vi "ZM-HWM-helperAcquisition.vi"(8 "error in":errorcluster, 10 "Event Registration Refnum":refnum<event-registration>, 11 "ZM-HWM-hardware_manager in":refnum<class "ZM-HWM-hardware_manager.lvclass">) -> (0 "error out":errorcluster)   [LabVIEW 2020, in "ZM-HWM-hardware_manager.lvlib" / "ZM-HWM-hardware_manager.lvclass"]
doc: "Helper loop of the hardware manager, started by Actor Core beside Call Parent. Every interval (ms) it reads the hardware (ZM-HW-do), sends the package to its actor and plots test packages on the chart. It stops on the actor's stop event or on an error; on an error it sends Normal Stop to its own actor. Error-handling plan: none yet; an error stops this actor and, through its Last Ack, its caller."
uses:
  ZM-HWM-hardware_manager.lvclass
  ZM-HWM-hardware_manager.lvclass/ZM-HWM-hardware_manager.ctl
  common/ZM-PC-packages/ZM-PC-TP-test_package/ZM-PC-TP-test_package.lvclass
  common/ZM-CI-common_interfaces/ZM-CI-handlePackage Msg/ZM-CI-handlePackage Msg.lvclass
  <vilib>/ActorFramework/Stop Msg/Stop Msg.lvclass
  hardware/ZM-HW-hardware/ZM-HW-hardware/ZM-HW-hardware.lvclass
  <vilib>/ActorFramework/Message Enqueuer/Message Enqueuer.lvclass
  <vilib>/ActorFramework/Actor/Actor.lvclass
panel:
  out "interval measured (ms)":u32
  in  "interval set (ms)":u32=500
  out "live":cluster{"temperature_c":dbl, "duty_percent":dbl}(graph)
  in  "stop":bool
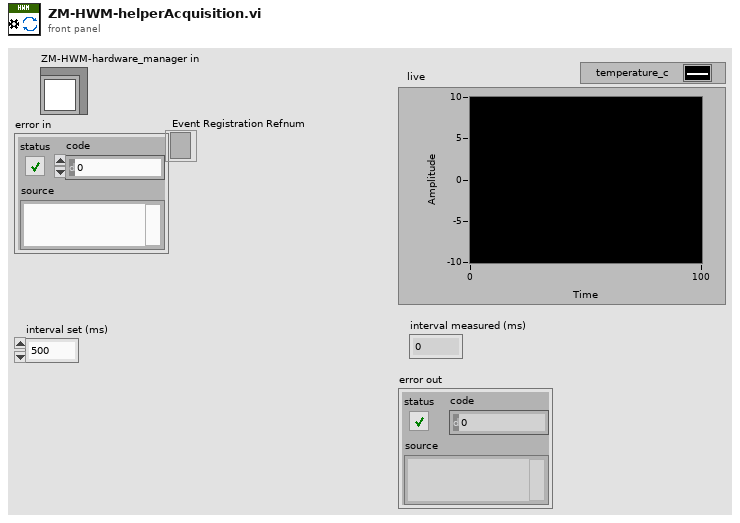
[diagram p1: front panel]
types:
  T1 = typedef "ZM-HWM-hardware_manager.lvlib/ZM-HWM-hardware_manager.lvclass/ZM-HWM-PRELAUNCH_SETTINGS.ctl" = cluster{"hardware":refnum<class "ZM-HW-hardware.lvclass">, "intervalMs":u32}
  T2 = typedef "ZM-PC-packages.lvlib/ZM-PC-TP-test_package.lvclass/ZM-PC-TP-DATA.ctl" = cluster{"temperature_c":dbl, "sample_index":i32, "duty_percent":u8, "sensor_ok":bool, "status":string}
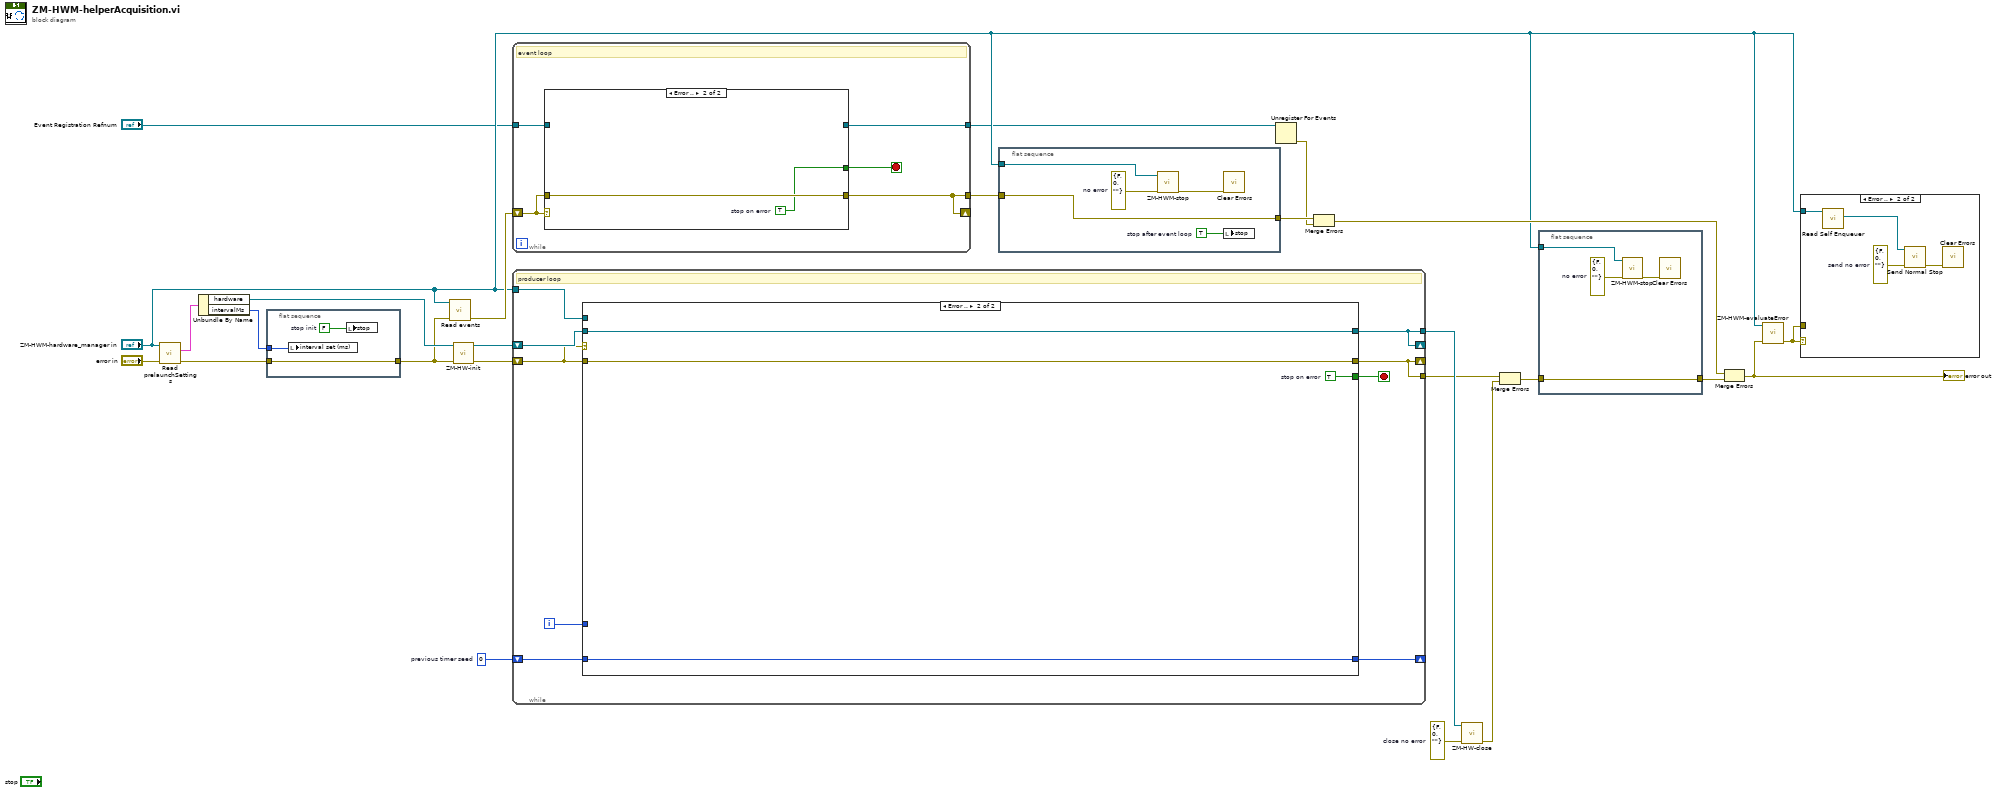
[diagram p0: block diagram]
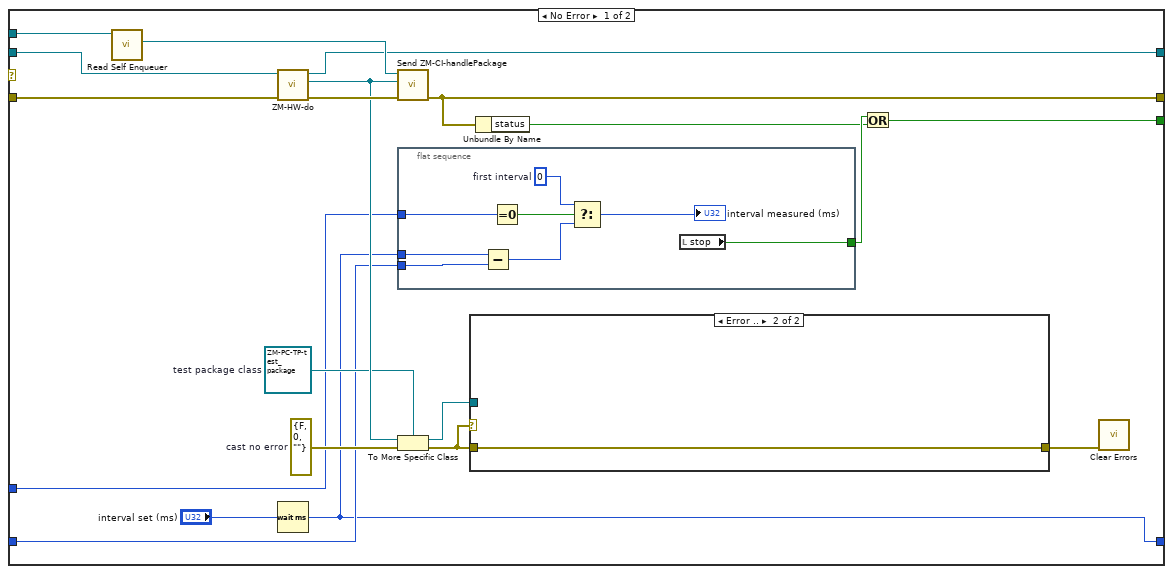
[diagram p3: hidden frame]
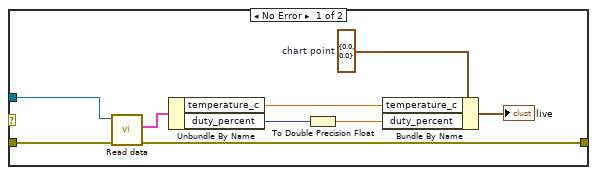
[diagram p4: hidden frame]
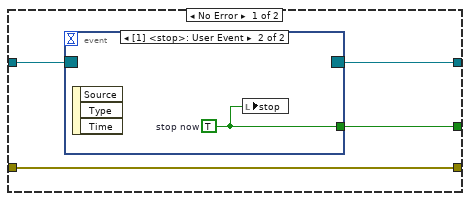
[diagram p5: hidden frame]
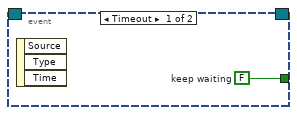
[diagram p6: hidden frame]
diagram:
  w11 = errorcluster {"status"=FALSE, "code"=0, "source"=""}  # close no error
  w13 = u32 0  # previous timer seed
  n1 = call "Read prelaunchSettings.vi"("error in (no error)"="error in", "ZM-HWM-hardware_manager in"="ZM-HWM-hardware_manager in") -> ("error out"=w23:errorcluster, "ZM-HWM-PRELAUNCH_SETTINGS"=w24:T1)  [unwired: 7 in, 1 out]
  n2 = Unbundle By Name(w24) -> ("hardware"=w21:refnum<class "ZM-HW-hardware.lvclass">, "intervalMs"=w22:u32)
  n3 = flat-sequence {
    tunnel: w23 -> [w26]
    tunnel: w22 -> [w27]
    tunnel: [w26] -> w20
    frame #0 {
      w28 = FALSE  # stop init
      n4 = local write "interval set (ms)"(w27) -> ()
      n5 = local write "stop"(w28) -> ()
    }
  }
  n6 = call "Read events.vi"("error in (no error)"=w20, "ZM-HWM-hardware_manager in"="ZM-HWM-hardware_manager in") -> ("error out"=w19:errorcluster)  [unwired: 7 in, 2 out]
  n7 = call-dynamic "ZM-HW-init.vi"("error in (no error)"=w20, "ZM-HW-hardware in"=w21) -> ("error out"=w15:errorcluster, "ZM-HW-hardware out"=w14:refnum<class "ZM-HW-hardware.lvclass">)  [unwired: 8 in]
  n8 = while {
    shift-right: [w31] -> _
    shift-left: w19 -> [w33]
    tunnel: [w31] -> w18
    tunnel: "Event Registration Refnum" -> [w30]
    tunnel: [w29] -> w2
    stop <- w32 stop-if-true
    # "event loop"
    n9 = case shown="Error .." w33 {
      tunnel: w33 -> [w37 w41]
      tunnel: [w37 w41] -> w31
      tunnel: [w36 w40] -> w32
      tunnel: w30 -> [w35 _]
      tunnel: [w34 _] -> w29
      frame No Error {
        n10 = event shown="[1] <stop>: User Event" {
          selector: w35 -> [_ _]
          dyn-events: [_ _] -> w34
          timeout: _ -> [_ _]
          tunnel: [w38 w39] -> w36
          event Timeout {
            w38 = FALSE  # keep waiting
            n11 = event-data() -> ()  [unwired: 1 in, 3 out]
          }
          event User Event {
            w39 = TRUE  # stop now
            n12 = event-data() -> ()  [unwired: 1 in, 3 out]
            n13 = local write "stop"(w39) -> ()
          }
        }
      }
      frame Error {
        w40 = TRUE  # stop on error
      }
    }
  }
  n14 = while {
    tunnel: "ZM-HWM-hardware_manager in" -> [w49]
    shift-right: [w44] -> _
    shift-left: w15 -> [w46]
    shift-right: [w43] -> _
    shift-left: w14 -> [w50]
    shift-right: [w47] -> _
    shift-left: w13 -> [w48]
    tunnel: [w44] -> w10
    tunnel: [w43] -> w12
    i -> [w42]
    stop <- w45 stop-if-true
    # "producer loop"
    n15 = case shown="Error .." w46 {
      tunnel: w46 -> [w69 w92]
      tunnel: w50 -> [w70 w91]
      tunnel: w49 -> [w68 _]
      tunnel: w48 -> [w58 w90]
      tunnel: w42 -> [w57 _]
      tunnel: [w54 w92] -> w44
      tunnel: [w53 w91] -> w43
      tunnel: [w52 w90] -> w47
      tunnel: [w51 w89] -> w45
      frame No Error {
        w64 = errorcluster {"status"=FALSE, "code"=0, "source"=""}  # cast no error
        w63 = refnum<class "ZM-PC-TP-test_package.lvclass"> refnum  # test package class
        n16 = call <vilib>:"Read Self Enqueuer.vi"("Actor"=w68) -> ("Self Enqueuer"=w67:refnum<class "Message Enqueuer.lvclass">)  [unwired: 10 in]
        n17 = call-dynamic "ZM-HW-do.vi"("error in (no error)"=w69, "ZM-HW-hardware in"=w70) -> ("error out"=w66:errorcluster, "package"=w65:refnum<class "ZM-PC-package.lvclass">, "ZM-HW-hardware out"=w53:refnum<class "ZM-HW-hardware.lvclass">)  [unwired: 7 in]
        n18 = Wait (ms)(milliseconds to wait="interval set (ms)") -> (millisecond timer value=w52:u32)
        n19 = call "Send ZM-CI-handlePackage.vi"("error in (no error)"=w66, "package"=w65, "Message Enqueuer"=w67) -> ("error out"=w54:errorcluster)  [unwired: 7 in, 1 out]
        n20 = flat-sequence {
          tunnel: w52 -> [w78]
          tunnel: w58 -> [w77]
          tunnel: w57 -> [w76]
          tunnel: [w71] -> w56
          frame #0 {
            w75 = u32 0  # first interval
            n21 = Subtract(x=w78, y=w77) -> (x-y=w73:u32)
            n22 = Equal To 0?(x=w76) -> (x = 0?=w74:bool)
            n23 = Select(t=w75, s=w74, f=w73) -> (s? t:f=→"interval measured (ms)":u32)
            n24 = local read "stop"() -> (w71:bool)
          }
        }
        n25 = To More Specific Class(target class=w63, reference=w65, error in=w64) -> (specific class reference=w62:refnum<class "ZM-PC-TP-test_package.lvclass">, error out=w61:errorcluster)
        n26 = case shown="Error .." w61 {
          tunnel: w62 -> [w86 _]
          tunnel: w61 -> [w87 w88]
          tunnel: [w79 w88] -> w60
          frame No Error {
            w81 = cluster{"temperature_c":dbl, "duty_percent":dbl} {"temperature_c"=0.0, "duty_percent"=0.0}  # chart point
            n27 = call "Read data.vi"("error in (no error)"=w87, "ZM-PC-TP-test_package in"=w86) -> ("error out"=w79:errorcluster, "ZM-PC-TP-DATA"=w85:T2)  [unwired: 7 in, 1 out]
            n28 = Unbundle By Name(w85) -> ("temperature_c"=w83:dbl, "duty_percent"=w84:u8)
            n29 = To Double Precision Float(number=w84) -> (double precision float=w82:dbl)
            n30 = Bundle By Name(cluster=w81, "temperature_c"=w83, "duty_percent"=w82) -> (→"live":cluster{"temperature_c":dbl, "duty_percent":dbl})
          }
          frame Error {
          }
        }
        n31 = Unbundle By Name(w54) -> ("status"=w55:bool)
        n32 = Or(x=w56, y=w55) -> (x .or. y?=w51:bool)
        n33 = call <vilib>:"Clear Errors.vi"("error in (no error)"=w60) -> ()  [unwired: 5 in, 2 out]
      }
      frame Error {
        w89 = TRUE  # stop on error
      }
    }
  }
  n34 = flat-sequence {
    tunnel: w18 -> [w93]
    tunnel: "ZM-HWM-hardware_manager in" -> [w96]
    tunnel: [w93] -> w17
    frame #0 {
      w95 = errorcluster {"status"=FALSE, "code"=0, "source"=""}  # no error
      w97 = TRUE  # stop after event loop
      n35 = call "ZM-HWM-stop.vi"("error in (no error)"=w95, "ZM-HWM-hardware_manager in"=w96) -> ("error out"=w94:errorcluster)  [unwired: 8 in, 1 out]
      n36 = call <vilib>:"Clear Errors.vi"("error in (no error)"=w94) -> ()  [unwired: 5 in, 2 out]
      n37 = local write "stop"(w97) -> ()
    }
  }
  n38 = Unregister For Events(event registration refnum=w2) -> (error out=w16:errorcluster)  [unwired: 1 in]
  n39 = Merge Errors(w17, w16) -> (w7:errorcluster)
  n40 = call-dynamic "ZM-HW-close.vi"("error in (no error)"=w11, "ZM-HW-hardware in"=w12) -> ("error out"=w9:errorcluster)  [unwired: 8 in, 1 out]
  n41 = Merge Errors(w10, w9) -> (w8:errorcluster)
  n42 = flat-sequence {
    tunnel: w8 -> [w98]
    tunnel: "ZM-HWM-hardware_manager in" -> [w101]
    tunnel: [w98] -> w6
    frame #0 {
      w100 = errorcluster {"status"=FALSE, "code"=0, "source"=""}  # no error
      n43 = call "ZM-HWM-stop.vi"("error in (no error)"=w100, "ZM-HWM-hardware_manager in"=w101) -> ("error out"=w99:errorcluster)  [unwired: 8 in, 1 out]
      n44 = call <vilib>:"Clear Errors.vi"("error in (no error)"=w99) -> ()  [unwired: 5 in, 2 out]
    }
  }
  n45 = Merge Errors(w7, w6) -> (w3:errorcluster)
  "error out" <- w3
  n46 = call "ZM-HWM-evaluateError.vi"("error in (no error)"=w3, "ZM-HWM-hardware_manager in"="ZM-HWM-hardware_manager in") -> ("error out"=w4:errorcluster)  [unwired: 7 in, 2 out]
  n47 = case shown="Error .." w4 {
    tunnel: w4 -> [_ _]
    tunnel: "ZM-HWM-hardware_manager in" -> [_ w105]
    frame No Error {
    }
    frame Error {
      w104 = errorcluster {"status"=FALSE, "code"=0, "source"=""}  # send no error
      n48 = call <vilib>:"Read Self Enqueuer.vi"("Actor"=w105) -> ("Self Enqueuer"=w103:refnum<class "Message Enqueuer.lvclass">)  [unwired: 10 in]
      n49 = call <vilib>:"Send Normal Stop.vi"("error in (no error)"=w104, "Message Enqueuer"=w103) -> ("error out"=w102:errorcluster)  [unwired: 9 in]
      n50 = call <vilib>:"Clear Errors.vi"("error in (no error)"=w102) -> ()  [unwired: 5 in, 2 out]
    }
  }
